vi "Close.vi"(8 "error in (no error)":errorcluster, 11 "Elevator in":refnum<class "Elevator.lvclass">) -> (0 "error out":errorcluster, 3 "Elevator out":refnum<class "Elevator.lvclass">)   [LabVIEW 2021, in "Elevator.lvclass"]
uses:
  Elevator.lvclass
  Elevator.lvclass/Elevator.ctl
  AnalogInput/AnalogInput.lvclass
  AnalogOutput/AnalogOutput.lvclass
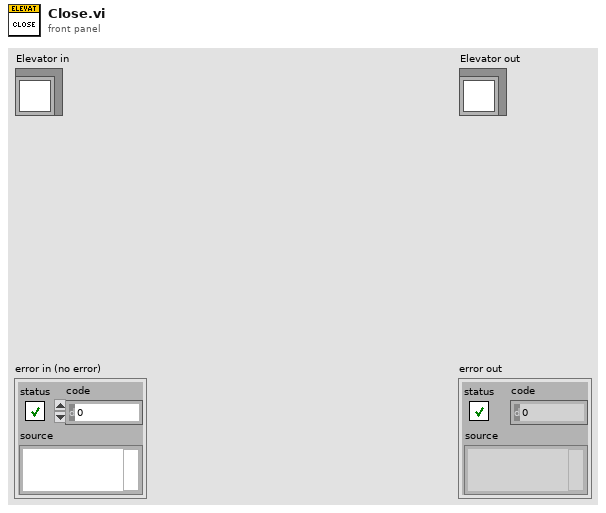
[diagram p1: front panel]
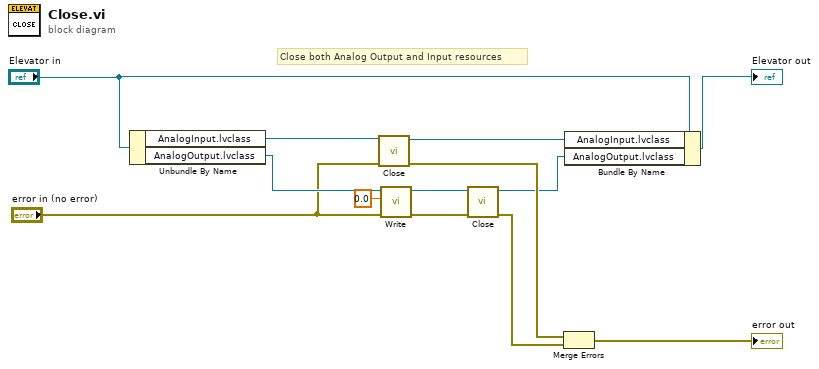
[diagram p0: block diagram]
diagram:
  # "Close both Analog Output and Input resources"
  n1 = Unbundle By Name("Elevator in") -> ("AnalogInput.lvclass"=w13:refnum<class "AnalogInput.lvclass">, "AnalogOutput.lvclass"=w8:refnum<class "AnalogOutput.lvclass">)
  n2 = call-dynamic "Close.vi"("error in (no error)"="error in (no error)", "AnalogInput in"=w13) -> ("error out"=w11:errorcluster, "AnalogInput out"=w10:refnum<class "AnalogInput.lvclass">)  [unwired: 8 in]
  n3 = call-dynamic "Write.vi"("error in (no error)"="error in (no error)", "data in"=0.0, "AnalogOutput in"=w8) -> ("error out"=w6:errorcluster, "AnalogOutput out"=w7:refnum<class "AnalogOutput.lvclass">)  [unwired: 7 in]
  n4 = call-dynamic "Close.vi"("error in (no error)"=w6, "AnalogOutput in"=w7) -> ("error out"=w12:errorcluster, "AnalogOutput out"=w9:refnum<class "AnalogOutput.lvclass">)  [unwired: 8 in]
  n5 = Merge Errors(w11, w12) -> (→"error out":errorcluster)
  n6 = Bundle By Name(cluster="Elevator in", "AnalogInput.lvclass"=w10, "AnalogOutput.lvclass"=w9) -> (→"Elevator out":refnum<class "Elevator.lvclass">)
